vi "Scaling_Parameters.vi"(8 "error in (no error)":errorcluster, 9 "Command Scale":cluster{"Output_Gain":dbl, "Output_Offset":dbl}={"Output_Gain"=1.0, "Output_Offset"=0.0}, 10 "Feedback Scale":cluster{"Input_Gain":dbl, "Input_Offset":dbl}={"Input_Gain"=1.0, "Input_Offset"=0.0}, 11 "Motor in":refnum<class "Motor.lvclass">) -> (0 "error out":errorcluster, 3 "Motor out":refnum<class "Motor.lvclass">)   [LabVIEW 2021, in "Motor.lvclass"]
uses:
  Motor.lvclass
  Motor.lvclass/Motor.ctl
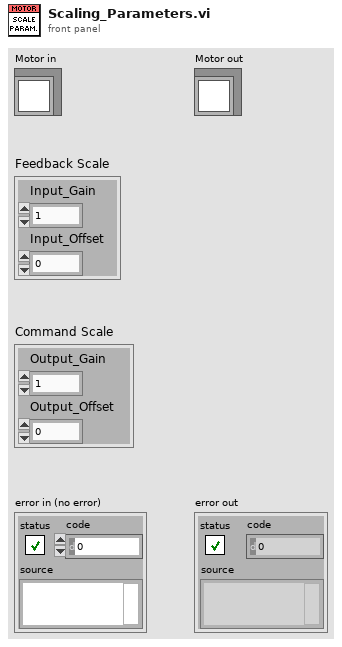
[diagram p1: front panel]
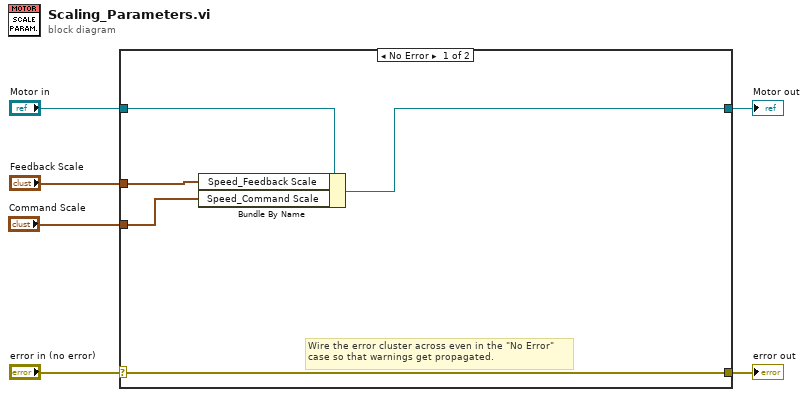
[diagram p0: block diagram]
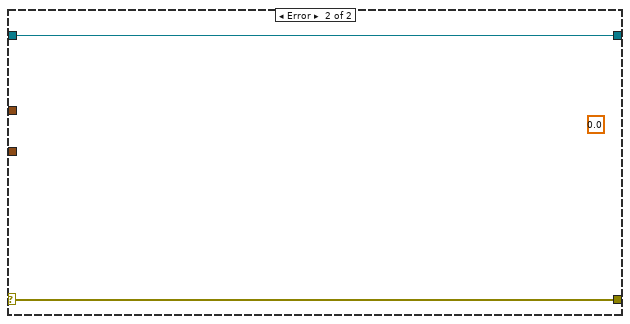
[diagram p2: hidden frame]
diagram:
  n1 = case shown="No Error" "error in (no error)" {
    selector: "error in (no error)" -> [w11 w13]
    tunnel: [w11 w13] -> w5
    tunnel: [w7 w12] -> w3
    tunnel: "Motor in" -> [w8 w12]
    tunnel: "Feedback Scale" -> [w10 _]
    tunnel: "Command Scale" -> [w9 _]
    frame No Error {
      # "Wire the error cluster across even in the \"No Error\"\ncase so that warnings get propagated."
      n2 = Bundle By Name(cluster=w8, "Speed_Feedback Scale"=w10, "Speed_Command Scale"=w9) -> (w7:refnum<class "Motor.lvclass">)
    }
    frame Error {
      (unwired) 0.0
    }
  }
  "error out" <- w5
  "Motor out" <- w3
